vi "Set ADC Number.vi"(8 "error in (no error)":errorcluster, 10 "ADC Number":T1=-1, 11 "CTI_AnalogIn in":refnum<class "CTI_AnalogIn.lvclass">) -> (0 "error out":errorcluster, 3 "CTI_AnalogIn out":refnum<class "CTI_AnalogIn.lvclass">)   [LabVIEW 2021, in "CTI_AnalogIn.lvclass"]
uses:
  CTI_AnalogIn.lvclass
  <vilib>/CTI/CTI Drivers/CTI/ADC Number.ctl
  CTI_AnalogIn.lvclass/CTI_AnalogIn.ctl
  <vilib>/CTI/CTI Drivers/CTI/CTI.lvlib
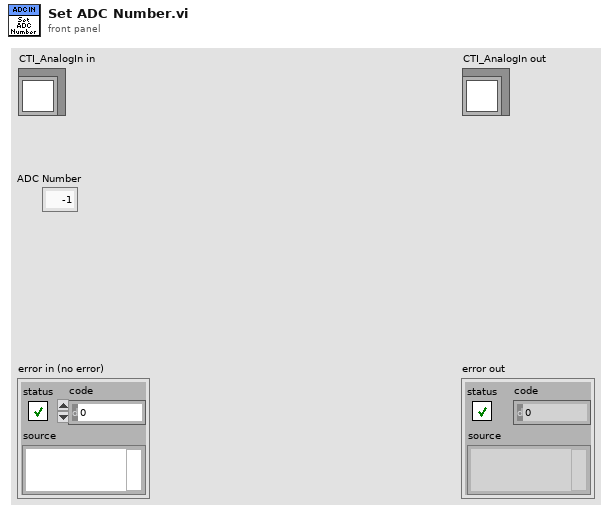
[diagram p1: front panel]
types:
  T1 = typedef "CTI.lvlib/ADC Number.ctl" = i8
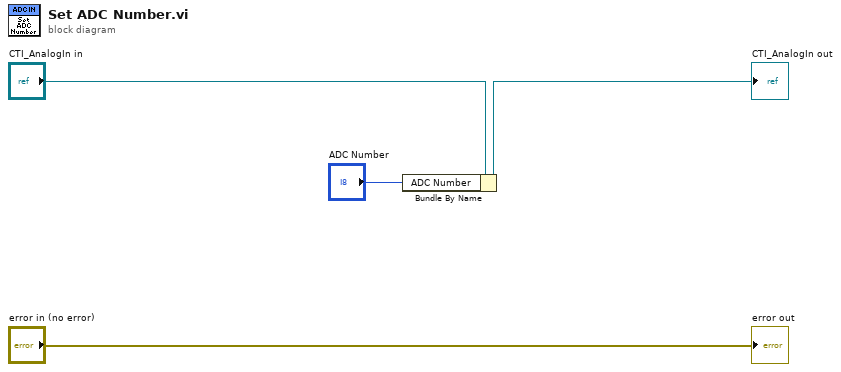
[diagram p0: block diagram]
diagram:
  n1 = Bundle By Name(cluster="CTI_AnalogIn in", "ADC Number"="ADC Number") -> (→"CTI_AnalogIn out":refnum<class "CTI_AnalogIn.lvclass">)
  "error out" <- "error in (no error)"
